vi "ReadStatus.vi"(7 "模块路径":path, 9 "sn":u16, 10 "错误输入（无错误）":errorcluster, 11 "会话句柄输入":refnum<k35>) -> (0 "Enable Sine Out":bool, 1 "Enable Profile ASF":bool, 2 "错误输出":errorcluster, 3 "会话句柄输出":refnum<k35>, 4 "Enable RAM":bool)   [LabVIEW 2018]
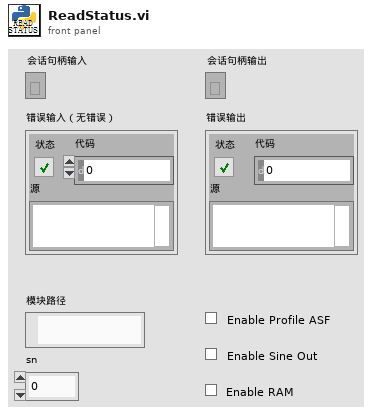
[diagram p1: front panel]
types:
  T1 = cluster{"Boolean array[0]":bool, "Boolean array[1]":bool, "Boolean array[2]":bool, "Boolean array[3]":bool, "Boolean array[4]":bool, "Boolean array[5]":bool, "Boolean array[6]":bool, "Boolean array[7]":bool}
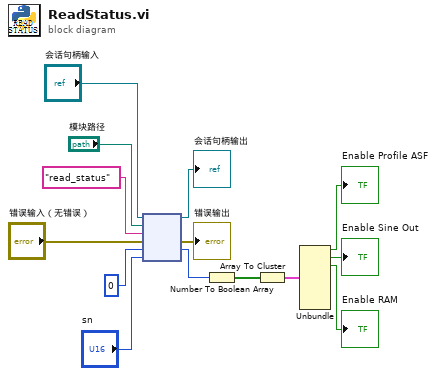
[diagram p0: block diagram]
diagram:
  n1 = node("会话句柄输入", "模块路径", "read_status", "错误输入（无错误）", u8 0, "sn") -> (→"会话句柄输出":refnum<k35>, →"错误输出":errorcluster, w7:u8)  [unwired: 1 in, 2 out]
  n2 = Number To Boolean Array(number=w7) -> (Boolean array=w6:bool[])
  n3 = Array To Cluster(array=w6) -> (cluster=w5:T1)
  n4 = Unbundle(w5) -> ("Boolean array[0]"=→"Enable Profile ASF":bool, "Boolean array[1]"=→"Enable Sine Out":bool, "Boolean array[2]"=→"Enable RAM":bool)  [unwired: 5 out]
